vi "VIH HelpGen - Build - Menus.vi"(8 "error in":errorcluster, 9 "File paths":path[](array[path]), 10 "Items":T2, 11 "Project Tree":T1) -> (0 "error out":errorcluster, 2 "Items out":T2, 3 "dup Project Tree":T1)   [LabVIEW 2014]
doc: "::: VI Helpeks :::\nCopyright (c) 2000-2026 Konstantin Shifershteyn. All rights reserved."
uses:
  _VIH Project Manager.llb/VIH Project Tree Typedef - Tree Refnum.ctl
panel:
  # "VI Helpeks\nCopyright (c) 2012-2026 Konstantin Shifershteyn"
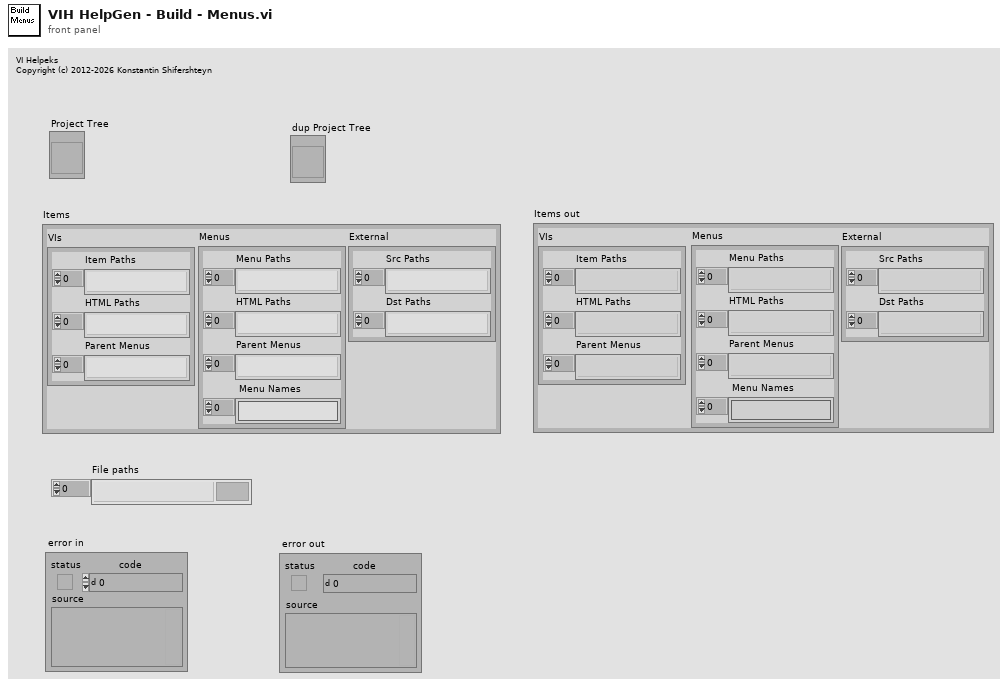
[diagram p1: front panel]
types:
  T1 = typedef "VIH Project Tree Typedef - Tree Refnum.ctl" = refnum<vi>
  T2 = cluster{"VIs":cluster{"Item Paths":path[], "HTML Paths":path[], "Parent Menus":path[]}, "Menus":cluster{"Menu Paths":path[], "HTML Paths":path[], "Parent Menus":path[], " Menu Names":string[]}, "External":cluster{"Src Paths":path[], "Dst Paths":path[]}}
  T3 = enum16{"nop", "Start", "Stop", "Run-prep", "Run-VI", "Run-Menu"}
  T4 = cluster{"Item Paths":path[], "HTML Paths":path[], "Parent Menus":path[]}
  T5 = cluster{"Menu Paths":path[], "HTML Paths":path[], "Parent Menus":path[], " Menu Names":string[]}
  T6 = cluster{"VIs":cluster{"Item Paths":path[], "HTML Paths":path[], "Parent Menus":path[]}, "Menus":cluster{"Menu Paths":path[], "HTML Paths":path[], "Parent Menus":path[], " Menu Names":string[]}}
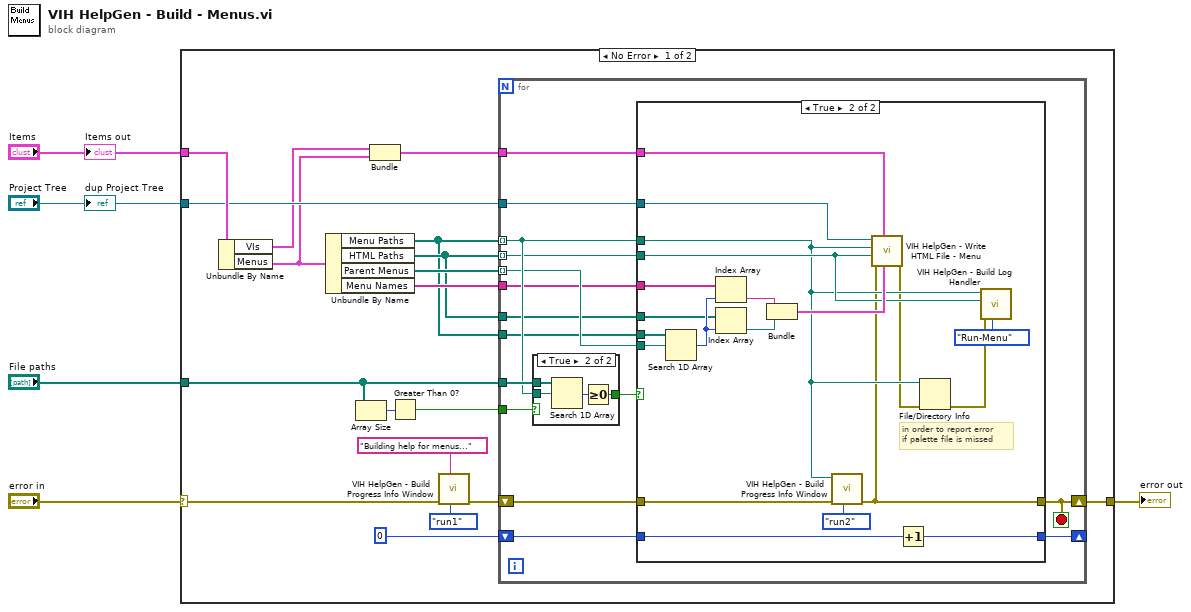
[diagram p0: block diagram]
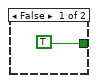
[diagram p3: hidden frame]
diagram:
  n1 = case shown="No Error" "error in" {
    selector: "error in" -> [w9 w66]
    tunnel: [w23 w66] -> w5
    tunnel: "Items" -> [w19 _]
    tunnel: "File paths" -> [w17 _]
    tunnel: "Project Tree" -> [w10 _]
    frame No Error {
      n2 = Unbundle By Name(w19) -> ("VIs"=w8:T4, "Menus"=w7:T5)
      n3 = Unbundle By Name(w7) -> ("Menu Paths"=w11:path[], "HTML Paths"=w20:path[], "Parent Menus"=w22:path[], "Menu Names"=w21:string[])
      n4 = Array Size(array=w17) -> (size(s)=w12:i32)
      n5 = Bundle("VIs"=w8, "Menus"=w7) -> (w6:T6)  [unwired: 1 in]
      n6 = Greater Than 0?(x=w12) -> (x > 0?=w13:bool)
      n7 = call "VIH HelpGen - Build Progress Info Window.vi"("Mode (run1)"=enum16{"start", "stop", "run1", "run2"}."run1" ("Mode (run)"), "Message"="Building help for menus...", "error in"=w9) -> ("error out"=w14:errorcluster)  [unwired: 8 in]
      n8 = for {
        tunnel: w13 -> [w38]
        tunnel: w17 -> [w37]
        tunnel: w11 -> [w35] mode=indexing
        tunnel: w20 -> [w34] mode=indexing
        shift-right: [w24] -> w23
        shift-left: w14 -> [w33]
        tunnel: w22 -> [w32] mode=indexing
        tunnel: w11 -> [w31]
        tunnel: w21 -> [w30]
        tunnel: w20 -> [w29]
        tunnel: w6 -> [w28]
        shift-right: [w26] -> _
        shift-left: 0 -> [w27]
        tunnel: w10 -> [w25]
        stop <- w24 stop-if-true
        n9 = case shown="True" w38 {
          tunnel: w37 -> [_ w65]
          tunnel: w35 -> [_ w64]
          tunnel: [TRUE w62] -> w36
          frame False {
          }
          frame True {
            n10 = Search 1D Array(1D array=w65, element=w64) -> (index of element=w63:i32)  [unwired: 1 in]
            n11 = Greater Or Equal To 0?(x=w63) -> (x >= 0?=w62:bool)
          }
        }
        n12 = case shown="True" w36 {
          tunnel: w35 -> [_ w44]
          tunnel: w34 -> [_ w45]
          tunnel: w33 -> [w40 w52]
          tunnel: [w40 w43] -> w24
          tunnel: w32 -> [_ w60]
          tunnel: w31 -> [_ w59]
          tunnel: w30 -> [_ w57]
          tunnel: w29 -> [_ w56]
          tunnel: w28 -> [_ w46]
          tunnel: w27 -> [w39 w51]
          tunnel: [w39 w50] -> w26
          tunnel: w25 -> [_ w48]
          frame False {
          }
          frame True {
            # "in order to report error\nif palette file is missed"
            n13 = Search 1D Array(1D array=w59, element=w60) -> (index of element=w58:i32)  [unwired: 1 in]
            n14 = Index Array(array=w57, index=w58) -> (element=w55:string)
            n15 = Index Array(array=w56, index=w58) -> (element=w54:path)
            n16 = Bundle("String"=w55, "Path"=w54) -> (w49:cluster{"String":string, "Path":path})  [unwired: 1 in]
            n17 = call "VIH HelpGen - Build Progress Info Window.vi"("Mode (run1)"=enum16{"start", "stop", "run1", "run2"}."run2" ("Mode (run)"), "error in"=w52, "Cur path"=w44) -> ("error out"=w43:errorcluster)  [unwired: 8 in]
            n18 = call "VIH HelpGen - Write HTML File - Menu.vi"("Owning Palette"=w49, "Items"=w46, "error in"=w43, "HTML Path"=w45, "Menu Path"=w44, "Project Tree"=w48) -> ("error out"=w42:errorcluster)  [unwired: 4 in, 1 out]
            n19 = Increment(x=w51) -> (x+1=w50:i32)
            n20 = File/Directory Info(path=w44, error in=w42) -> (error out=w41:errorcluster)  [unwired: 6 out]
            n21 = call "VIH HelpGen - Build Log Handler.vi"("cmd (nop)"=T3."Run-Menu" ("cmd"), "error in"=w41, "Out File Path"=w45, "Src File Path"=w44) -> ()  [unwired: 3 in, 5 out]
          }
        }
      }
    }
    frame Error {
    }
  }
  "error out" <- w5
  "Items out" <- "Items"
  "dup Project Tree" <- "Project Tree"
